vi "Write File (Complete).vi"(8 "error in (no error)":errorcluster, 10 "String":string, 11 "ConfigManager.Text in":refnum<class "ConfigManager.Text.lvclass">) -> (0 "error out":errorcluster, 3 "ConfigManager.Text out":refnum<class "ConfigManager.Text.lvclass">)   [LabVIEW 2013, in "CfgManager.Text.lvlib" / "ConfigManager.Text.lvclass"]
uses:
  ConfigManager.Text.lvclass
  Manager/ConfigManager.lvclass/ConfigManager.ctl
  Manager/ConfigManager.lvclass
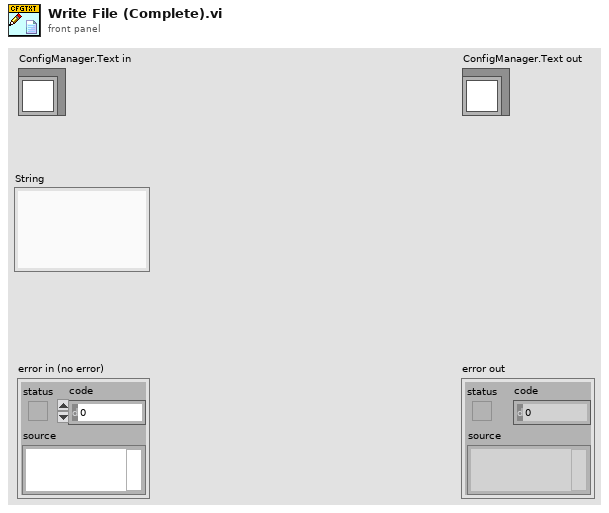
[diagram p1: front panel]
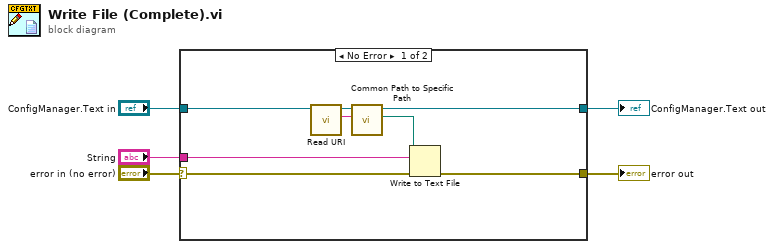
[diagram p0: block diagram]
diagram:
  n1 = case shown="No Error" "error in (no error)" {
    selector: "error in (no error)" -> [w12 w14]
    tunnel: [w11 w14] -> w4
    tunnel: [w8 w13] -> w2
    tunnel: "ConfigManager.Text in" -> [w9 w13]
    tunnel: "String" -> [w10 _]
    frame No Error {
      n2 = call "Read URI.vi"("ConfigManager in"=w9) -> ("URI"=w7:string, "ConfigManager out"=w8:refnum<class "ConfigManager.Text.lvclass">)  [unwired: 9 in]
      n3 = call "Common Path to Specific Path.vi"("common path"=w7) -> ("specific path"=w6:path)  [unwired: 10 in]
      n4 = Write to Text File(file (use dialog)=w6, text=w10, error in=w12) -> (error out=w11:errorcluster)  [unwired: 1 in, 2 out]
    }
    frame Error {
    }
  }
  "error out" <- w4
  "ConfigManager.Text out" <- w2
